vi "Set Icons.vi"() -> ()   [LabVIEW 2020]
doc: "Development tool: sets the icons of many VIs at once and saves each one. VIs and Icons are text files with the paths of the VIs and of their 32x32 PNGs, in the same order, separated by semicolons (written by tools/dev/icons.py). Opens each VI, sets its icon from the file, saves it and closes the reference; codes has one error code per VI (0 = done). Run it with no project open; a VI that is running or has unsaved changes cannot be saved."
panel:
  out "error out":errorcluster
  out "codes":i32[](array[numeric])
  in  "Icons":path
  in  "VIs":path
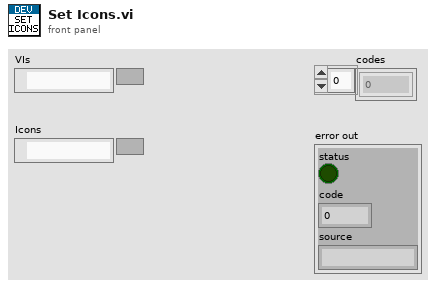
[diagram p1: front panel]
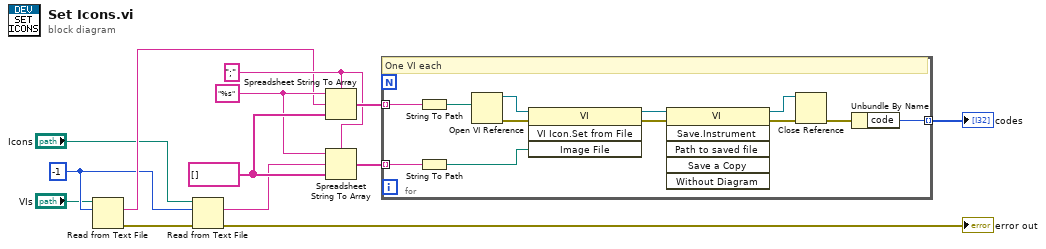
[diagram p0: block diagram]
diagram:
  w10 = ";"
  w9 = string[] []
  w8 = "%s"
  w3 = -1
  n1 = Read from Text File(file (use dialog)="VIs", count=w3) -> (text=w4:string, error out=w5:errorcluster)  [unwired: 2 in, 2 out]
  n2 = Read from Text File(file (use dialog)="Icons", count=w3, error in=w5) -> (text=w6:string, error out=→"error out":errorcluster)  [unwired: 1 in, 2 out]
  n3 = Spreadsheet String To Array(delimiter (Tab)=w10, format string=w8, spreadsheet string=w4, array type (2D Dbl)=w9) -> (array=w11:string[])
  n4 = Spreadsheet String To Array(delimiter (Tab)=w10, format string=w8, spreadsheet string=w6, array type (2D Dbl)=w9) -> (array=w12:string[])
  n5 = for {
    tunnel: w11 -> [w14] mode=indexing
    tunnel: w12 -> [w15] mode=indexing
    tunnel: [w25] -> w13 mode=indexing
    # "One VI each"
    n6 = String To Path(string=w14) -> (path=w16:path)
    n7 = String To Path(string=w15) -> (path=w17:path)
    n8 = Open VI Reference(vi path=w16) -> (vi reference=w18:refnum<vi>, error out=w19:errorcluster)  [unwired: 5 in]
    n9 = invoke class="VI" method="VI Icon.Set from File"(reference=w18, error in=w19, "Image File"=w17) -> (reference out=w20:refnum<vi>, error out=w21:errorcluster)  [unwired: 1 in, 2 out]
    n10 = invoke class="VI" method="Save.Instrument"(reference=w20, error in=w21) -> (reference out=w22:refnum<vi>, error out=w23:errorcluster)  [unwired: 4 in, 4 out]
    n11 = Close Reference(reference=w22, error in (no error)=w23) -> (error out=w24:errorcluster)
    n12 = Unbundle By Name(w24) -> ("code"=w25:i32)
  }
  "codes" <- w13
